vi "Init.vi"(7 "I2C #":T2=-1, 8 "error in (no error)":errorcluster, 9 "Address":T1=57 format="%02x", 10 "Session In":refnum<class "Session.lvclass">) -> (0 "error out":errorcluster, 3 "AS7431 Light Spectrum Out":refnum<class "AS7431 11 Ch Light Spectrum Sensor.lvclass">)   [LabVIEW 2020, in "CTI-Peripheral.lvlib" / "AS7431 11 Ch Light Spectrum Sensor.lvclass"]
uses:
  AS7431 11 Ch Light Spectrum Sensor.lvclass
  CTI/Session/Session.lvclass
  CTI/I2C Number.ctl
  CTI/I2C Address.ctl
  CTI/I2C Connection/I2C Connection.lvclass/I2C Connection.ctl
  AS7431 11 Ch Light Spectrum Sensor.lvclass/AS7431 11 Ch Light Spectrum Sensor.ctl
  CTI/I2C Connection/I2C Connection.lvclass
  CTI/CTI.lvlib
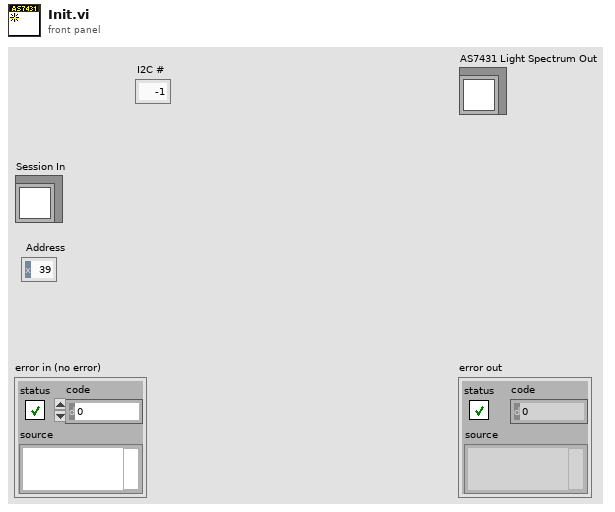
[diagram p1: front panel]
types:
  T1 = typedef "CTI.lvlib/I2C Address.ctl" = u8
  T2 = typedef "CTI.lvlib/I2C Number.ctl" = i8
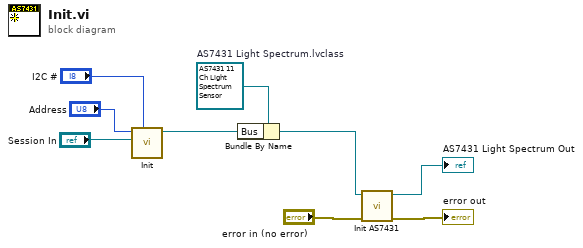
[diagram p0: block diagram]
diagram:
  w5 = refnum<class "AS7431 11 Ch Light Spectrum Sensor.lvclass"> refnum  # AS7431 Light Spectrum.lvclass
  n1 = call "Init.vi"("I2C #"="I2C #", "Session"="Session In", "Address"="Address") -> ("I2C Connection"=w9:refnum<class "I2C Connection.lvclass">)  [unwired: 7 in, 1 out]
  n2 = Bundle By Name(cluster=w5, "Bus"=w9) -> (w4:refnum<class "AS7431 11 Ch Light Spectrum Sensor.lvclass">)
  n3 = call "Init AS7431.vi"("error in (no error)"="error in (no error)", "ADS1115 in"=w4) -> ("error out"=→"error out":errorcluster, "ADS1115 out"=→"AS7431 Light Spectrum Out":refnum<class "AS7431 11 Ch Light Spectrum Sensor.lvclass">)  [unwired: 8 in]
